vi "_Publish DP Indicators(VI).vi"(7 "VIRef(Caller VI)/RefMgr":refnum<vi>, 8 "error in (no error)":errorcluster, 9 "force update(F)":bool, 11 "SILAPI In":refnum<k1>) -> (0 "error out":errorcluster, 1 "Binded DPs":string[](array[string]), 3 "SILAPI Out":refnum<k1>)   [LabVIEW 2017, in "TagDB RefManager.lvlib"]
uses:
  TagDB RefManager.lvlib
  10d0bc68-ff5b-4b3e-94b6-72122e87f5c0.vi
  99199be5-3273-4500-92d5-279e96ad7927.vi
  936e1e9c-d5b6-4b4e-ad99-7c7dab878fa3.vi
  12cc79ca-27a7-4410-b99e-89b61dace636.vi
  <userlib>/_NEVSTOP/TagDB/_Support/DataAccess/_NameCacher.vi
  <userlib>/_NEVSTOP/TagDB/_Support/Error/_[error50002]Invalid DataType.vi
  <userlib>/_NEVSTOP/TagDB/_Support/Error/_[error50000]Invalid DB REF.vi
  <userlib>/_NEVSTOP/TagDB/_Support/DataAccess/TagDB Ref to DVR.vi
  <userlib>/_NEVSTOP/TagDB/_Support/URL/TRIM-BOTH-SPACE.vi
  <userlib>/_NEVSTOP/TagDB/_Support/Error/_Build Error Cluster.vi
  <userlib>/_NEVSTOP/TagDB/TagDB.lvlib
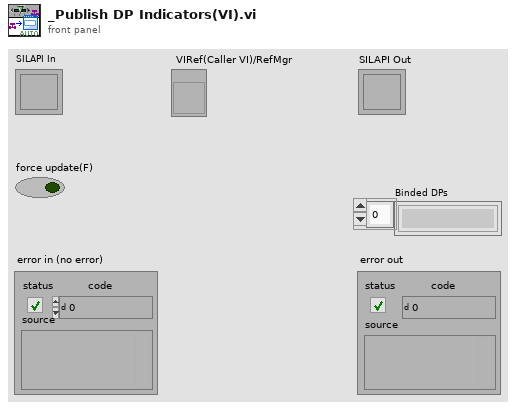
[diagram p1: front panel]
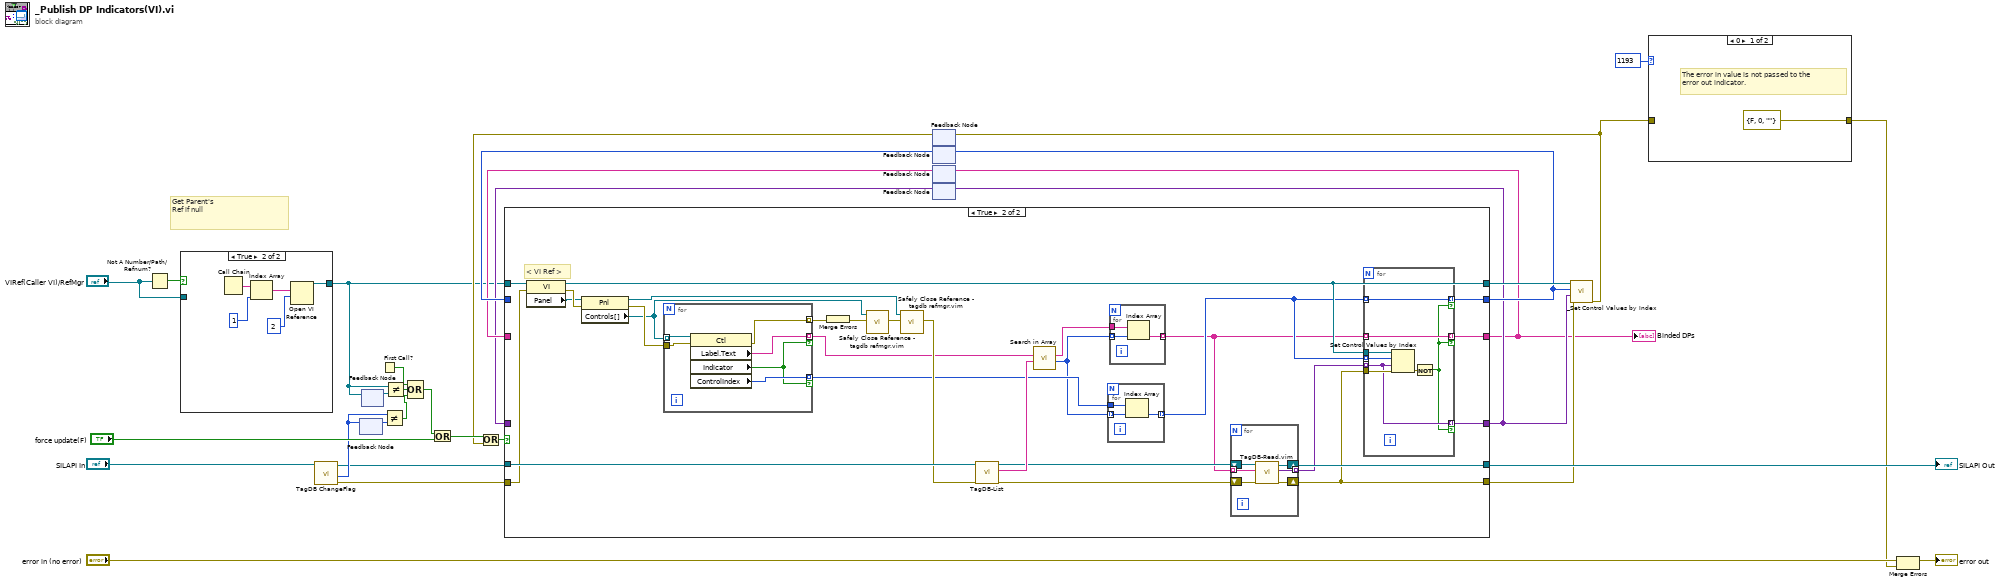
[diagram p0: block diagram]
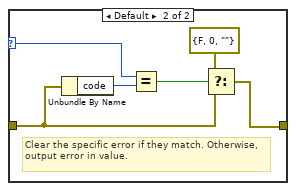
[diagram p2: hidden frame]
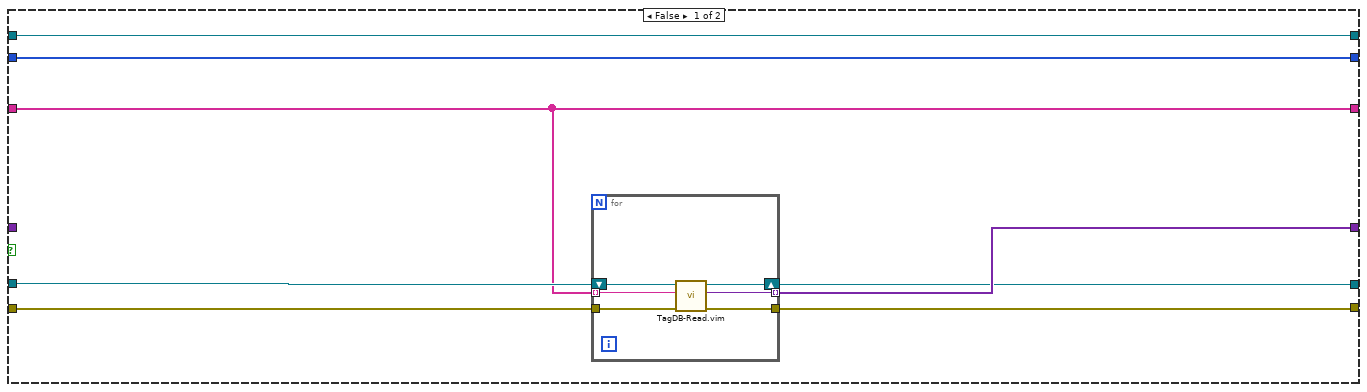
[diagram p3: hidden frame]
diagram:
  # "Get Parent's\nRef if null"
  n1 = Not A Number/Path/Refnum?(number/path/refnum="VIRef(Caller VI)/RefMgr") -> (NaN/Path/Refnum?=w12:bool)
  n2 = case shown="True" w12 {
    tunnel: [w32 w33] -> w8
    tunnel: "VIRef(Caller VI)/RefMgr" -> [w32 _]
    frame False {
    }
    frame True {
      n3 = Call Chain() -> (call chain=w37:string[])
      n4 = Index Array(array=w37, index=1 ("Index")) -> (element=w35:string)
      n5 = Open VI Reference(vi path=w35, options=2) -> (vi reference=w33:refnum<vi>)  [unwired: 4 in, 1 out]
    }
  }
  n6 = call <userlib>:"TagDB ChangeFlag.vi"("DB Ref"="SILAPI In") -> ("error in (no error) (dup)"=w1:errorcluster, "Item Change Timestamp"=w5:u64, "DB Ref (dup)"=w3:refnum<k1>)  [unwired: 7 in, 1 out]
  n7 = feedback #1() -> (w6:u64)  [unwired: 1 in]
  n8 = feedback-in #1(w5) -> ()
  n9 = feedback #2() -> (w11:refnum<vi>)  [unwired: 1 in]
  n10 = feedback-in #2(w8) -> ()
  n11 = First Call?() -> (First Call?: T/F=w9:bool)
  n12 = Not Equal?(x=w5, y=w6) -> (x != y?=w2:bool)
  n13 = Not Equal?(x=w8, y=w11) -> (x != y?=w10:bool)
  n14 = Compound Arithmetic op=OR(w9, w10, w2) -> (w7:bool)
  n15 = Or(x=w7, y="force update(F)") -> (x .or. y?=w23:bool)
  n16 = feedback #3() -> (w14:errorcluster)  [unwired: 1 in]
  n17 = Or(x=w23, y=w14) -> (x .or. y?=w16:bool)
  n18 = feedback #4() -> (w24:i32[])  [unwired: 1 in]
  n19 = feedback #5() -> (w22:string[])  [unwired: 1 in]
  n20 = feedback #6() -> (w19:variant[])  [unwired: 1 in]
  n21 = case shown="True" w16 {
    tunnel: [w45 w68] -> w26
    tunnel: w8 -> [w45 w79]
    tunnel: [w44 w72] -> w25
    tunnel: w24 -> [w44 _]
    tunnel: [w42 w73] -> w17
    tunnel: w22 -> [w42 _]
    tunnel: [w40 w71] -> w20
    tunnel: w3 -> [w43 w78]
    tunnel: [w41 w74] -> w21
    tunnel: w19 -> [_ _]
    tunnel: [w39 w76] -> w27
    tunnel: w1 -> [w38 w52]
    frame False {
      n22 = for {
        tunnel: w42 -> [w50] mode=indexing
        tunnel: [w49] -> w41
        tunnel: [w48] -> w40 mode=indexing
        shift-right: [w47] -> w39
        shift-left: w43 -> [w51]
        tunnel: w38 -> [w46]
        n23 = call "TagDB-Read.vim"("error in (no error)"=w46, "name"=w50, "TagDB"=w51) -> ("error out"=w49:errorcluster, "Value"=w48:variant, "TagDB(dup)"=w47:refnum<k1>)  [unwired: 3 in, 3 out]
      }
    }
    frame True {
      # "< VI Ref >"
      n24 = property class="VI"(reference=w79, error in=w52) -> (reference out=w68:refnum<vi>, error out=w70:errorcluster, "Panel"=w69:refnum<vi>)
      n25 = property class="Pnl"(reference=w69, error in=w70) -> (reference out=w60:refnum<vi>, error out=w66:errorcluster, "Controls[]"=w61:refnum<vi>[])
      n26 = for {
        tunnel: w61 -> [w97] mode=indexing
        tunnel: [w96] -> w55 mode=indexing if=w94
        tunnel: [w95] -> w58 mode=indexing if=w94
        tunnel: [w93] -> w67 mode=indexing
        tunnel: w66 -> [w92]
        n27 = property class="Ctl"(reference=w97, error in=w92) -> (error out=w93:errorcluster, "Label.Text"=w96:string, "Indicator"=w94:bool, "ControlIndex"=w95:i32)  [unwired: 1 out]
      }
      n28 = Merge Errors(w67) -> (w62:errorcluster)
      n29 = call "Safely Close Reference - tagdb refmgr.vim"("error in (no error)"=w62, "Reference"=w61) -> ("error out"=w63:errorcluster)  [unwired: 9 in]
      n30 = call "Safely Close Reference - tagdb refmgr.vim"("error in (no error)"=w63, "Reference"=w60) -> ("error out"=w59:errorcluster)  [unwired: 9 in]
      n31 = call <userlib>:"TagDB-List.vi"("error in (no error)"=w59, "TagDB"=w78) -> ("error out"=w77:errorcluster, "names"=w65:string[], "TagDB(dup)"=w64:refnum<k1>)  [unwired: 6 in, 1 out]
      n32 = call "Search in Array.vi"("items to filter"=w65, "array"=w55) -> ("item Indexs"=w56:i32[], "array(dup)"=w53:string[])  [unwired: 4 in]
      n33 = for {
        tunnel: w56 -> [w85] mode=indexing
        tunnel: w58 -> [w84]
        tunnel: [w83] -> w57 mode=indexing
        n34 = Index Array(array=w84, index=w85) -> (element=w83:i32)
      }
      n35 = for {
        tunnel: w56 -> [w82] mode=indexing
        tunnel: w53 -> [w81]
        tunnel: [w80] -> w54 mode=indexing
        n36 = Index Array(array=w81, index=w82) -> (element=w80:string)
      }
      n37 = for {
        tunnel: [w89] -> w75 mode=indexing
        tunnel: w54 -> [w87] mode=indexing
        shift-right: [w88] -> w74
        shift-left: w77 -> [w91]
        shift-right: [w90] -> w76
        shift-left: w64 -> [w86]
        n38 = call "TagDB-Read.vim"("error in (no error)"=w91, "name"=w87, "TagDB"=w86) -> ("error out"=w88:errorcluster, "Value"=w89:variant, "TagDB(dup)"=w90:refnum<k1>)  [unwired: 3 in, 3 out]
      }
      n39 = for {
        tunnel: w68 -> [w105]
        tunnel: w57 -> [w104] mode=indexing
        tunnel: w75 -> [w100] mode=indexing
        tunnel: w74 -> [w103]
        tunnel: [w102] -> w73 mode=indexing if=w98
        tunnel: w54 -> [w102] mode=indexing
        tunnel: [w101] -> w72 mode=indexing if=w98
        tunnel: w57 -> [w101] mode=indexing
        tunnel: [w100] -> w71 mode=indexing if=w98
        n40 = Set Control Values by Index(0:w105, 1:w104, 2:w100, 3:w103) -> (11:w99:errorcluster)
        n41 = Not(x=w99) -> (.not. x?=w98:bool)
      }
    }
  }
  "SILAPI Out" <- w27
  "Binded DPs" <- w17
  n42 = feedback-in #4(w25) -> ()
  n43 = feedback-in #5(w17) -> ()
  n44 = feedback-in #6(w20) -> ()
  n45 = call <userlib>:"_Set Control Values by Index.vi"("error in (no error)"=w21, "data values"=w20, "control indexes"=w25, "VI Refnum"=w26) -> ("error out"=w15:errorcluster)  [unwired: 7 in]
  n46 = feedback-in #3(w15) -> ()
  n47 = case shown="0" 1193 ("specific error code to clear (0: all)") {
    selector: 1193 ("specific error code to clear (0: all)") -> [_ w111]
    tunnel: w15 -> [_ w110]
    tunnel: [errorcluster {"status"=FALSE, "code"=0, "source"=""} ("error constant") w107] -> w18
    frame 0 {
      # "The error in value is not passed to the\nerror out indicator."
    }
    frame Default {
      # "Clear the specific error if they match. Otherwise, output error in value."
      n48 = Unbundle By Name(w110) -> ("code"=w112:i32)
      n49 = Equal?(x=w111, y=w112) -> (x = y?=w108:bool)
      n50 = Select(t=errorcluster {"status"=FALSE, "code"=0, "source"=""} ("error constant"), s=w108, f=w110) -> (s? t:f=w107:errorcluster)
    }
  }
  n51 = Merge Errors("error in (no error)", w18) -> (→"error out":errorcluster)
